vi "Command.vi"(8 "error in (no error)":errorcluster, 10 "Http Chan Cmd":T1, 11 "HTTP Command Bridge in":refnum<class "HTTP Command Bridge.lvclass">) -> (0 "error out":errorcluster, 3 "HTTP Command Bridge out":refnum<class "HTTP Command Bridge.lvclass">)   [LabVIEW 2020, in "Volatus.lvlib" / "HTTP Command Bridge.lvclass"]
uses:
  HTTP Command Bridge.lvclass
  C:/dev/lv20CE/relink/lv-volatus/Volatus/Module/Module.lvclass
  Http Chan Cmd.ctl
  Http Cmd Type.ctl
  HTTP Command Bridge.lvclass/HTTP Command Bridge.ctl
  messages/CmdDigital/Data.ctl
  MessageQ/MessageQ.lvclass/MessageQ.ctl
  messages/CmdDigital/Class/Msg.lvclass/Msg.ctl
  Module/Module.lvclass/Module.ctl
  VolatusAPI/VolatusAPI.lvclass/VolatusAPI.ctl
  messages/CmdAnalog/Data.ctl
  messages/CmdAnalog/Class/Msg.lvclass/Msg.ctl
  messages/CmdDigital/Class/Msg.lvclass
  C:/dev/lv20CE/relink/lv-protoc/LV-Proto/Message/Message.lvclass
  messages/CmdAnalog/Class/Msg.lvclass
  lv-vecto/Vecto/TCPMessageService/Send Message.vi
  lv-protoc/LV-Proto/Message/Message.lvclass
  Module/Module.lvclass
  messages/CmdDigital/CmdDigital.lvlib
  VolatusAPI/VolatusAPI.lvclass
  MessageQ/MessageQ.lvclass
  messages/CmdAnalog/CmdAnalog.lvlib
  Volatus.lvlib
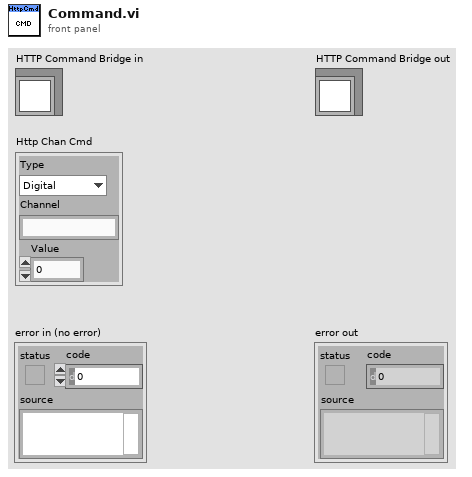
[diagram p1: front panel]
types:
  T1 = typedef "Volatus.lvlib/Http Chan Cmd.ctl" = cluster{"Type":T2, "Channel":string, "Value":dbl}
  T2 = typedef "Volatus.lvlib/Http Cmd Type.ctl" = enum16{"Digital", "Numeric"}
  T3 = typedef "Volatus.lvlib/HTTP Command Bridge.lvclass/Command Info.ctl" = cluster{"Destination":T4, "Local Q":refnum<class "MessageQ.lvclass">, "Target":string, "Task":string}
  T4 = typedef "Volatus.lvlib/HTTP Command Bridge.lvclass/Command Dest.ctl" = enum16{"Local", "Remote"}
  T5 = typedef "CmdDigital.lvlib/Data.ctl" = cluster{"channel":string, "value":bool}
  T6 = typedef "CmdAnalog.lvlib/Data.ctl" = cluster{"channel":string, "value":dbl}
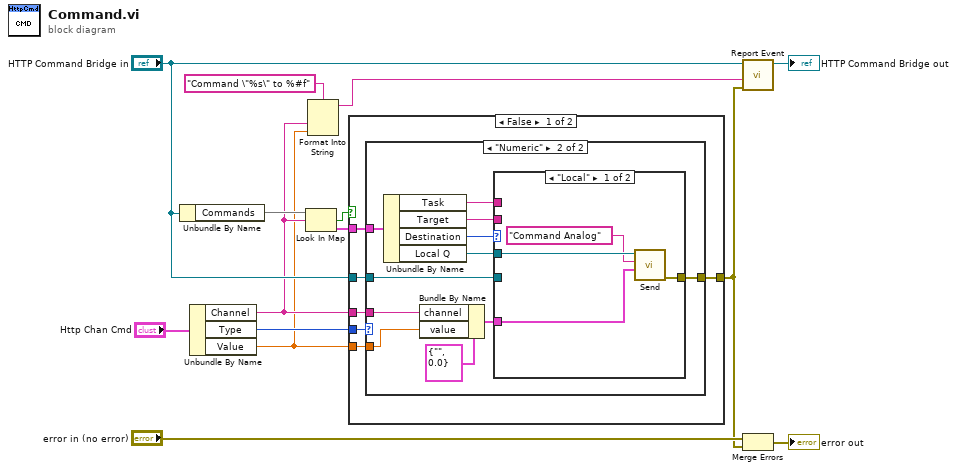
[diagram p0: block diagram]
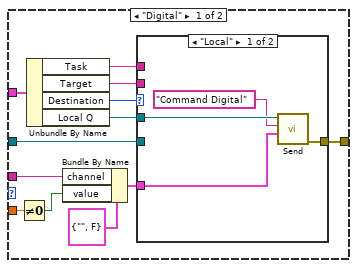
[diagram p2: hidden frame]
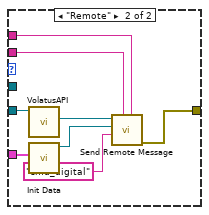
[diagram p3: hidden frame]
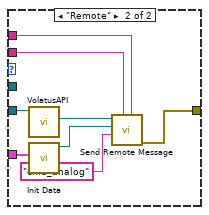
[diagram p4: hidden frame]
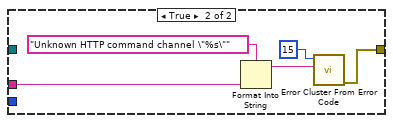
[diagram p5: hidden frame]
diagram:
  n1 = Unbundle By Name("HTTP Command Bridge in") -> ("Commands"=w13:map{string, T3})
  n2 = Unbundle By Name("Http Chan Cmd") -> ("Channel"=w4:string, "Type"=w9:T2, "Value"=w3:dbl)
  n3 = Look In Map(map=w13, key=w4) -> (key not found?=w11:bool, value=w10:T3)  [unwired: 1 in]
  n4 = Format Into String(format string="Command \"%s\" to %#f", w4, w3) -> (resulting string=w2:string)  [unwired: 2 in, 1 out]
  n5 = case shown="False" w11 {
    tunnel: w10 -> [w17 _]
    tunnel: w9 -> [w20 _]
    tunnel: w3 -> [w18 _]
    tunnel: w4 -> [w19 w68]
    tunnel: "HTTP Command Bridge in" -> [w16 _]
    tunnel: [w15 w72] -> w1
    frame False {
      n6 = case shown="\"Numeric\"" w20 {
        tunnel: w19 -> [w30 w53]
        tunnel: w18 -> [w29 w52]
        tunnel: w17 -> [w27 w51]
        tunnel: w16 -> [w22 w46]
        tunnel: [w21 w45] -> w15
        frame "Digital" {
          n7 = Not Equal To 0?(x=w29) -> (x != 0?=w28:bool)
          n8 = Unbundle By Name(w27) -> ("Task"=w23:string, "Target"=w24:string, "Destination"=w26:T4, "Local Q"=w25:refnum<class "MessageQ.lvclass">)
          n9 = Bundle By Name(cluster=T5 {"channel"="", "value"=FALSE} ("Data"), "channel"=w30, "value"=w28) -> (w31:T5)
          n10 = case shown="\"Local\"" w26 {
            tunnel: w31 -> [w34 w44]
            tunnel: w25 -> [w36 _]
            tunnel: w24 -> [_ w39]
            tunnel: w23 -> [_ w38]
            tunnel: w22 -> [_ w43]
            tunnel: [w33 w37] -> w21
            frame "Local" {
              n11 = call "Send.vi"("Data"=w34, "ID"="Command Digital", "MessageQ in"=w36) -> ("error out"=w33:errorcluster)  [unwired: 7 in, 1 out]
            }
            frame "Remote" {
              n12 = call "VolatusAPI.vi"("Module in"=w43) -> ("VolatusAPI"=w42:refnum<class "VolatusAPI.lvclass">)  [unwired: 9 in, 1 out]
              n13 = call "Init Data.vi"("Data"=w44) -> ("Msg out"=w41:refnum<class "Msg.lvclass">)  [unwired: 10 in]
              n14 = call "Send Remote Message.vi"("Target Task (None)"=w38, "Target Name"=w39, "Message Type"="cmd_digital", "Message"=w41, "VolatusAPI in"=w42) -> ("error out"=w37:errorcluster)  [unwired: 5 in, 1 out]
            }
          }
        }
        frame "Numeric" {
          n15 = Unbundle By Name(w51) -> ("Task"=w47:string, "Target"=w48:string, "Destination"=w50:T4, "Local Q"=w49:refnum<class "MessageQ.lvclass">)
          n16 = Bundle By Name(cluster=T6 {"channel"="", "value"=0.0} ("Data"), "channel"=w53, "value"=w52) -> (w54:T6)
          n17 = case shown="\"Local\"" w50 {
            tunnel: w54 -> [w57 w67]
            tunnel: w49 -> [w59 _]
            tunnel: w48 -> [_ w62]
            tunnel: w47 -> [_ w61]
            tunnel: w46 -> [_ w66]
            tunnel: [w56 w60] -> w45
            frame "Local" {
              n18 = call "Send.vi"("Data"=w57, "ID"="Command Analog", "MessageQ in"=w59) -> ("error out"=w56:errorcluster)  [unwired: 7 in, 1 out]
            }
            frame "Remote" {
              n19 = call "VolatusAPI.vi"("Module in"=w66) -> ("VolatusAPI"=w65:refnum<class "VolatusAPI.lvclass">)  [unwired: 9 in, 1 out]
              n20 = call "Init Data.vi"("Data"=w67) -> ("Msg out"=w64:refnum<class "Msg.lvclass">)  [unwired: 10 in]
              n21 = call "Send Remote Message.vi"("Target Task (None)"=w61, "Target Name"=w62, "Message Type"="cmd_analog", "Message"=w64, "VolatusAPI in"=w65) -> ("error out"=w60:errorcluster)  [unwired: 5 in, 1 out]
            }
          }
        }
      }
    }
    frame True {
      n22 = Format Into String(format string="Unknown HTTP command channel \"%s\"", w68) -> (resulting string=w70:string)  [unwired: 2 in, 1 out]
      n23 = call <vilib>:"Error Cluster From Error Code.vi"("error message (\"\")"=w70, "error code (0)"=15) -> ("error out"=w72:errorcluster)  [unwired: 7 in]
    }
  }
  n24 = call "Report Event.vi"("error in (no error)"=w1, "Message"=w2, "Module in"="HTTP Command Bridge in") -> ("Module out"=→"HTTP Command Bridge out":refnum<class "HTTP Command Bridge.lvclass">)  [unwired: 7 in, 1 out]
  n25 = Merge Errors("error in (no error)", w1) -> (→"error out":errorcluster)
